vi "Snapshot_Run.vi"(11 "error in":errorcluster) -> ()   [LabVIEW 2026]
doc: "Test of the whole picture build-up: Test_Setup, then Ticks ticks of Game_Step with the key script (At, Key), each tick drawn by Frame_Draw (the whole screen) and rastered. The screen after the last tick is saved as Resources\\Preview\\<File name>. Avg ms / Max ms = time of Frame_Draw."
uses:
  Source/Render/GH_Render.lvlib
  Source/Engine/GH_Engine.lvlib
  Source/Level/GH_Level.lvlib
panel:
  out "error out":errorcluster
  out "Max ms":u32
  out "Avg ms":dbl
  in  "Keys":i32
  in  "File name":string="lv_run.png"
  in  "Phase":i32=2
  in  "Torch":bool
  in  "Y":i32
  in  "X":i32
  in  "Room":i32=-1
  in  "Level":i32=1
  in  "Ticks":i32=60
  in  "Key":u16[](array[numeric])
  in  "At":i32[](array[numeric])
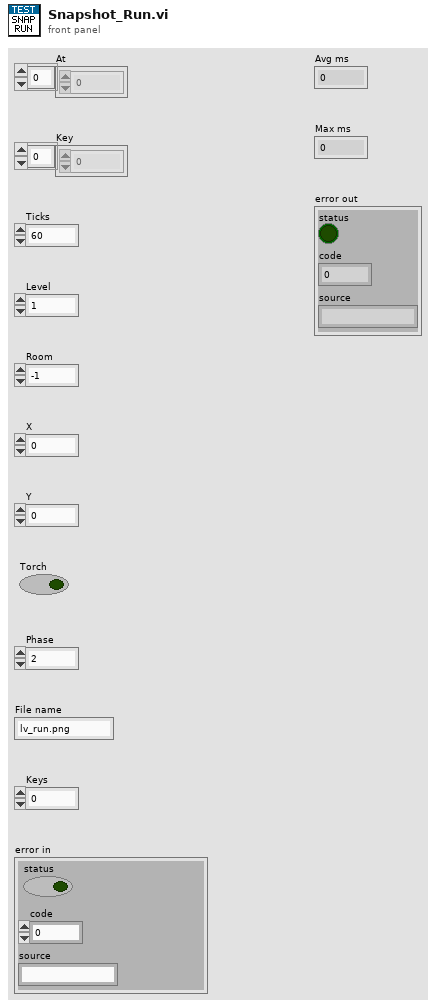
[diagram p1: front panel]
types:
  T1 = cluster{"RoomKey":i32, "Key":i32, "NameKey":i32, "Lit":u8[][], "Dim":u8[][], "Dark":u8[][], "Comp":u8[][], "Template":cluster{"image type":i32, "image depth":i32, "image":u8[], "mask":u8[], "colors":u32[], "Rectangle":cluster{"left":i16, "top":i16, "right":i16, "bottom":i16}}, "CX":i32, "CY":i32, "X1":i32, "Y1":i32, "X2":i32, "Y2":i32, "Prev":cluster{"Kind":i32, "X10":i32, "Y10":i32, "Dir":i32, "Mode":i32}[], "HudKey":i32, "HudScore":i32, "HudTime":i32, "Full":cluster{"image type":i32, "image depth":i32, "image":u8[], "mask":u8[], "colors":u32[], "Rectangle":cluster{"left":i16, "top":i16, "right":i16, "bottom":i16}}[]}
  T2 = cluster{"image type":i32, "image depth":i32, "image":u8[], "mask":u8[], "colors":u32[], "Rectangle":cluster{"left":i16, "top":i16, "right":i16, "bottom":i16}}
  T3 = cluster{"Tick":u32, "Phase":i32, "PhaseTicks":i32, "Level":i32, "Room":i32, "X10":i32, "Y10":i32, "VY10":i32, "Mode":i32, "Facing":i32, "Run":i32, "Vert":i32, "StandY":i32, "EntryX10":i32, "EntryY10":i32, "EntryMode":i32, "Lives":i32, "Score":i32, "NextLife":i32, "KeyR":i32, "KeyB":i32, "KeyY":i32, "Torch":bool, "FloorPhase":i32, "Dead":bool, "LevelStart":bool, "Quit":bool, "Sound":i32, "Seed":u32, "DemoStep":i32, "Tiles":u8[][], "World":cluster{"ID":string, "Depth":i32, "Column":i32, "Tiles":u8[][]}[], "Enemies":cluster{"Kind":i32, "X10":i32, "Y10":i32, "Dir":i32, "Mode":i32}[], "Highscores":cluster{"Score":i32, "Name":string}[], "Name":i32[], "Cursor":i32}
  T4 = cluster{"ID":string, "Depth":i32, "Column":i32, "Tiles":u8[][]}[]
  T5 = cluster{"left":i16, "top":i16, "right":i16, "bottom":i16}
  T6 = typedef "imagedata.ctl" = cluster{"image type":i32, "image depth":i32, "image":u8[], "mask":u8[], "colors":u32[], "Rectangle":cluster{"left":i16, "top":i16, "right":i16, "bottom":i16}}
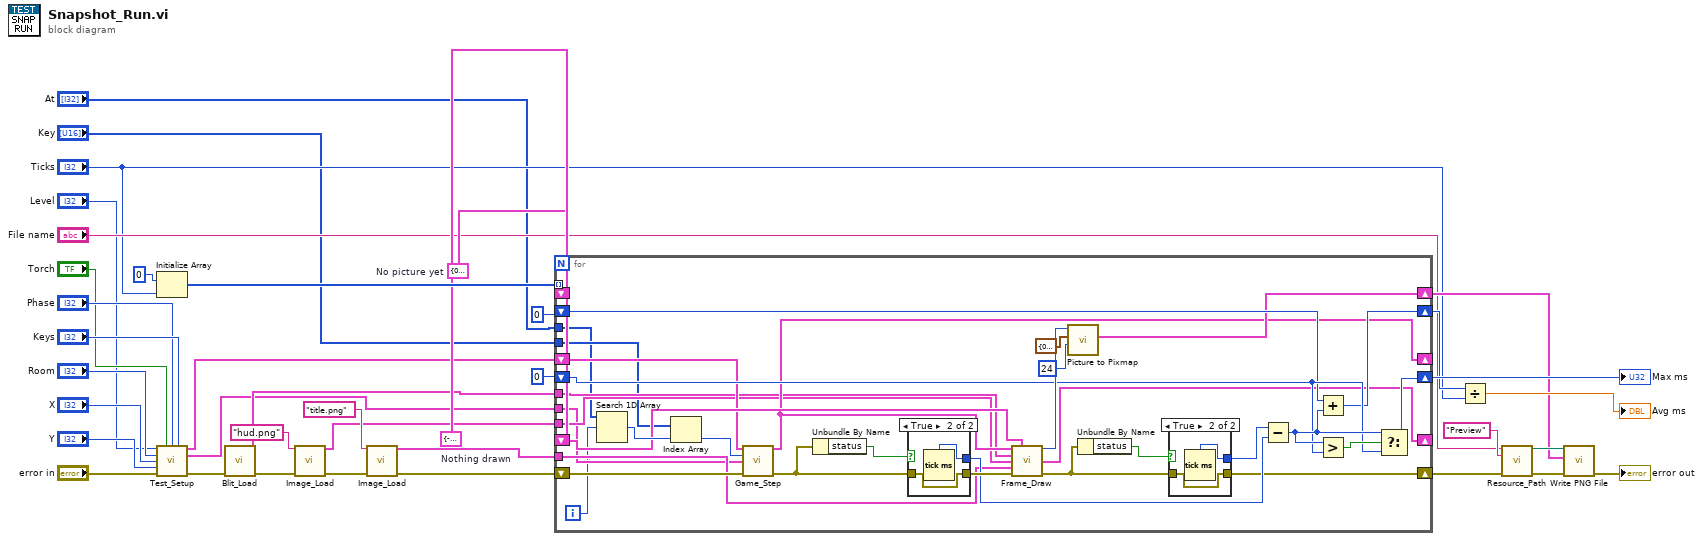
[diagram p0: block diagram]
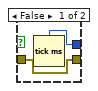
[diagram p2: hidden frame]
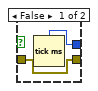
[diagram p3: hidden frame]
diagram:
  w25 = T1 {"RoomKey"=-1, "Key"=-1, "NameKey"=-1, "Lit"=[], "Dim"=[], "Dark"=[], "Comp"=[], "Template"={"image type"=0, "image depth"=0, "image"=[], "mask"=[], "colors"=[], "Rectangle"={"left"=0, "top"=0, "right"=0, "bottom"=0}}, "CX"=-1, "CY"=-1, "X1"=0, "Y1"=0, "X2"=0, "Y2"=0, "Prev"=[], "HudKey"=-1, "HudScore"=-1, "HudTime"=-1, "Full"=[]}  # Nothing drawn
  w24 = T2 {"image type"=0, "image depth"=0, "image"=[], "mask"=[], "colors"=[], "Rectangle"={"left"=0, "top"=0, "right"=0, "bottom"=0}}  # No picture yet
  n1 = Initialize Array(0, "Ticks") -> (w29:i32[])
  n2 = call "Test_Setup.vi"("Level"="Level", "Torch"="Torch", "Phase"="Phase", "Keys"="Keys", "Room"="Room", "X"="X", "Y"="Y", "error in"="error in") -> ("State"=w13:T3, "Rooms"=w14:T4, "error out"=w15:errorcluster)  [unwired: 5 in]
  n3 = call "Blit_Load.vi"("error in"=w15) -> ("Sprites"=w16:cluster{"Pix":u8[][], "Mask":u8[][]}[], "error out"=w17:errorcluster)  [unwired: 13 in]
  n4 = call "Image_Load.vi"("File name"="hud.png", "error in"=w17) -> ("Image"=w19:T2, "error out"=w20:errorcluster)  [unwired: 12 in]
  n5 = call "Image_Load.vi"("File name"="title.png", "error in"=w20) -> ("Image"=w22:T2, "error out"=w23:errorcluster)  [unwired: 12 in]
  n6 = for {
    tunnel: "At" -> [w40]
    tunnel: "Key" -> [w41]
    shift-right: [w51] -> _
    shift-left: w25 -> [w50]
    shift-right: [w52] -> w31
    shift-left: w24 -> [_]
    shift-right: [w54] -> w32
    shift-left: u32 0 -> [w53]
    shift-right: [w56] -> w33
    shift-left: u32 0 -> [w55]
    tunnel: w29 -> [_] mode=indexing
    tunnel: w14 -> [w42]
    shift-right: [w47] -> _
    shift-left: w13 -> [w46]
    tunnel: w16 -> [w43]
    tunnel: w19 -> [w44]
    tunnel: w22 -> [w45]
    shift-right: [w49] -> w30
    shift-left: w23 -> [w48]
    i -> [w39]
    n7 = Search 1D Array(1D array=w40, element=w39) -> (index of element=w57:i32)  [unwired: 1 in]
    n8 = Index Array(array=w41, index=w57) -> (element=w58:u16)
    n9 = call "Game_Step.vi"("State"=w46, "Key"=w58, "Rooms"=w42, "error in"=w48) -> ("State out"=w47:T3, "error out"=w59:errorcluster)  [unwired: 10 in]
    n10 = Unbundle By Name(w59) -> ("status"=w60:bool)
    n11 = case shown="True" w60 {
      tunnel: [w76 w78] -> w61
      tunnel: w59 -> [w75 w77]
      tunnel: [w75 w77] -> w62
      frame False {
        n12 = Tick Count (ms)() -> (millisecond timer value=w76:u32)
      }
      frame True {
        n13 = Tick Count (ms)() -> (millisecond timer value=w78:u32)
      }
    }
    n14 = call "Frame_Draw.vi"("State"=w47, "Memory"=w50, "Sprites"=w43, "Hud"=w44, "Title"=w45, "error in"=w62) -> ("Picture"=w63:picture, "Memory out"=w51:T1, "error out"=w64:errorcluster)  [unwired: 6 in, 1 out]
    n15 = call <vilib>:"Picture to Pixmap.vi"("depth"=24, "rect"=T5 {"left"=0, "top"=0, "right"=1280, "bottom"=720}, "picture"=w63) -> ("image data"=w52:T6)  [unwired: 7 in, 1 out]
    n16 = Unbundle By Name(w64) -> ("status"=w65:bool)
    n17 = case shown="True" w65 {
      tunnel: [w72 w74] -> w66
      tunnel: w64 -> [w71 w73]
      tunnel: [w71 w73] -> w49
      frame False {
        n18 = Tick Count (ms)() -> (millisecond timer value=w72:u32)
      }
      frame True {
        n19 = Tick Count (ms)() -> (millisecond timer value=w74:u32)
      }
    }
    n20 = Subtract(x=w66, y=w61) -> (x-y=w67:u32)
    n21 = Add(x=w53, y=w67) -> (x+y=w54:u32)
    n22 = Greater?(x=w67, y=w55) -> (0:w70:bool)
    n23 = Select(t=w67, s=w70, f=w55) -> (s? t:f=w56:u32)
  }
  "Max ms" <- w33
  n24 = Divide(x=w32, y="Ticks") -> (x/y=→"Avg ms":dbl)
  n25 = call "Resource_Path.vi"("File name"="File name", "Subfolder"="Preview", "error in"=w30) -> ("Path"=w35:path, "error out"=w36:errorcluster)  [unwired: 11 in]
  n26 = call <vilib>:"Write PNG File.vi"("error in (no error)"=w36, "image data"=w31, "path to PNG file"=w35) -> ("error out"=→"error out":errorcluster)  [unwired: 7 in, 1 out]
